vi "Prepare Control.vi"(7 "VolatusAPI":refnum<class "VolatusAPI.lvclass">, 8 "error in (no error)":errorcluster, 11 "ValveControl in":refnum<class "InterlockControl.lvclass">) -> (0 "error out":errorcluster, 3 "ValveControl out":refnum<class "InterlockControl.lvclass">)   [LabVIEW 2020, in "VolatusControl.lvlib" / "InterlockControl.lvclass"]
uses:
  InterlockControl.lvclass
  Volatus/VolatusAPI/VolatusAPI.lvclass
  InterlockControl.lvclass/InterlockControl.ctl
  Volatus/VolatusAPI/VolatusAPI.lvclass/VolatusAPI.ctl
  Volatus/Module Identity/Module Identity.lvclass/Module Identity.ctl
  lv-vecto/Vecto/Channel DBL/Channel DBL.lvclass/Channel DBL.ctl
  Volatus/Module Identity/Create.vi
  Volatus/Module Identity/Module Identity.lvclass
  C:/dev/lv20CE/relink/lv-volatus/Volatus/Identity/Identity.lvclass
  lv-vecto/Vecto/ChannelService/Lookup Double Channel.vi
  lv-vecto/Vecto/Group DBL/Value by Index.vi
  Volatus/VolatusAPI/Lookup Channel Info.vi
  <vilib>/Utility/error.llb/Error Cluster From Error Code.vi
  Volatus/VolatusAPI/Lookup Q.vi
  Volatus/MessageQ/MessageQ.lvclass
  lv-vecto/Vecto/Channel DBL/Channel DBL.lvclass
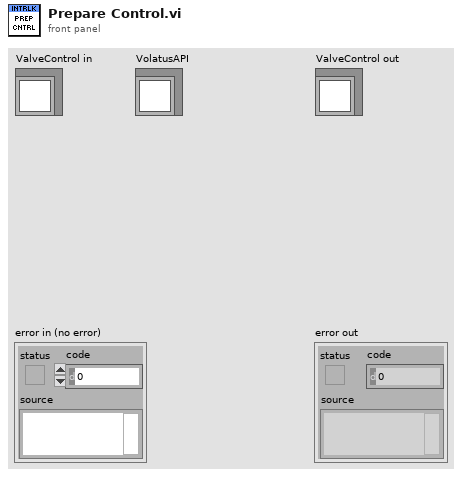
[diagram p1: front panel]
types:
  T1 = typedef "VolatusControl.lvlib/InterlockControl.lvclass/Inhibit Condition.ctl" = cluster{"Channel Name":string, "Comparison":T2, "Value":dbl}
  T2 = typedef "VolatusControl.lvlib/InterlockControl.lvclass/Inhibit Comparison.ctl" = enum16{"Equal", "Less Than", "Greater Than"}
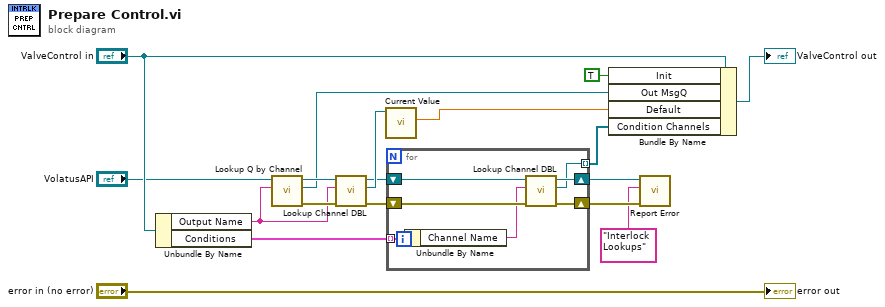
[diagram p0: block diagram]
diagram:
  n1 = Unbundle By Name("ValveControl in") -> ("Output Name"=w7:string, "Conditions"=w14:T1[])
  n2 = call "Lookup Q by Channel.vi"("Channel Name"=w7, "VolatusAPI in"="VolatusAPI") -> ("error out"=w18:errorcluster, "MessageQ"=w1:refnum<class "MessageQ.lvclass">, "VolatusAPI out"=w5:refnum<class "VolatusAPI.lvclass">)  [unwired: 7 in]
  n3 = call "Lookup Channel DBL.vi"("error in (no error)"=w18, "Name"=w7, "VolatusAPI in"=w5) -> ("error out"=w3:errorcluster, "Channel DBL"=w9:refnum<class "Channel DBL.lvclass">, "VolatusAPI out"=w4:refnum<class "VolatusAPI.lvclass">)  [unwired: 6 in]
  n4 = call "Current Value.vi"("Channel in"=w9) -> ("Scaled"=w2:dbl)  [unwired: 6 in, 4 out]
  n5 = for {
    tunnel: w14 -> [w23] mode=indexing
    tunnel: [w19] -> w13 mode=indexing
    shift-right: [w21] -> w11
    shift-left: w3 -> [w25]
    shift-right: [w20] -> w12
    shift-left: w4 -> [w24]
    n6 = Unbundle By Name(w23) -> ("Channel Name"=w22:string)
    n7 = call "Lookup Channel DBL.vi"("error in (no error)"=w25, "Name"=w22, "VolatusAPI in"=w24) -> ("error out"=w21:errorcluster, "Channel DBL"=w19:refnum<class "Channel DBL.lvclass">, "VolatusAPI out"=w20:refnum<class "VolatusAPI.lvclass">)  [unwired: 6 in]
  }
  n8 = Bundle By Name(cluster="ValveControl in", "Init"=TRUE, "Out MsgQ"=w1, "Default"=w2, "Condition Channels"=w13) -> (→"ValveControl out":refnum<class "InterlockControl.lvclass">)
  n9 = call "Report Error.vi"("error in (no error)"=w11, "Context"="Interlock Lookups", "VolatusAPI in"=w12) -> ()  [unwired: 7 in, 2 out]
  "error out" <- "error in (no error)"
